vi "KYFG Set Grabber Value.vi"(8 "error in (no error)":errorcluster, 9 "paramValue":i64, 10 "paramName":string, 11 "handle":u32) -> (0 "error out":errorcluster, 1 "paramValue out":i64, 3 "function return":u32(ring))   [LabVIEW 2023, in "KYFGLib_lv.lvlib"]
doc: "KYFG_API FGSTATUS KYFG_SetGrabberValue(FGHANDLE handle, const char *paramName, void *paramValue);"
uses:
  KYFGLib_lv.lvlib
  KYFGLib.dll
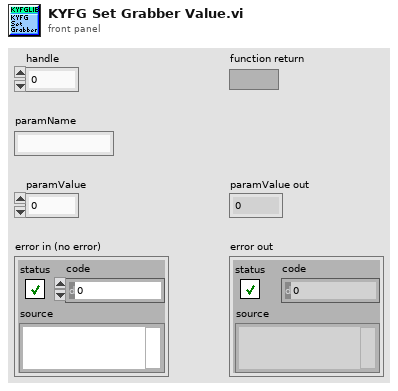
[diagram p1: front panel]
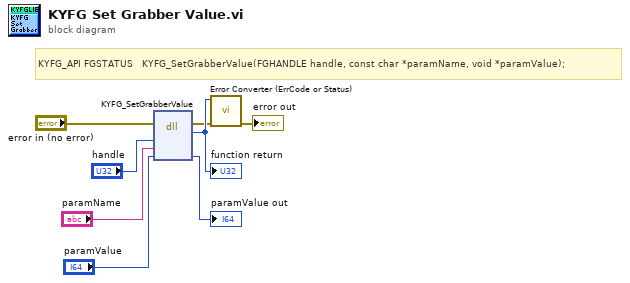
[diagram p0: block diagram]
diagram:
  # "KYFG_API FGSTATUS   KYFG_SetGrabberValue(FGHANDLE handle, const char *paramName, void *paramValue);"
  n1 = dll-call lib="KYFGLib.dll" fn="KYFG_SetGrabberValue"(error in="error in (no error)", "handle"="handle", "paramName"="paramName", "paramValue"="paramValue") -> (error out=w2:errorcluster, "return type"=w8:u32, "paramValue"=→"paramValue out":i64)  [unwired: 4 in, 1 out]
  "function return" <- w8
  n2 = call "Error Converter (ErrCode or Status).vi"("error in (no error)"=w2, "error code"=w8) -> ("error out"=→"error out":errorcluster)  [unwired: 9 in]
